vi "Initialize.vi"(6 "Filter":T1 {"Deny List (ID)" format="%.0x"; "Allow List (ID)" format="%.0x"}, 7 "Use OS Timestamp":bool, 8 "error in (no error)":errorcluster, 9 "Port Configuration":T2={"Mode"=enum."CAN FD", "Baud Rate"=500000, "Temination On"=TRUE, "Subordinate"=FALSE, "Echo TX"=FALSE, "FD Config"={"FD Baud Rate"=2000000, "ISO Mode"=TRUE, "BRS Enabled"=TRUE}} {"FD Config"."FD Baud Rate" format="%.0p"; "Baud Rate" format="%.0p"}, 10 "Interface":string, 11 "XNET_CAN_RW in":refnum<class "XNET CAN RW.lvclass">) -> (0 "error out":errorcluster, 3 "XNET_CAN_RW out":refnum<class "XNET CAN RW.lvclass">)   [LabVIEW 2021, in "XNET CAN RW.lvclass"]
doc: "Initialize a CAN read or write session using NI XNET hardware. \n\nInterface is the name of the XNET interface (eg CAN1)\n\nPort configuration sets the details of the CAN communication. Subordinate indicates another session has already configured the CAN port and this should use those settings.\n\nFilter provides a mecahnism to allow (white list) and deny (black list) certain ID from being returned or output. \n\nUse OS Timestamp will cause a read to replace the timestamp from the CAN driver with a timestamp from the OS. This is useful for correlation to othe events on the OS since the CAN clock will drift from the OS clock."
uses:
  XNET CAN RW.lvclass
  C:/Program Files/National Instruments/LabVIEW 2021/vi.lib/CIF Foundation/CIF CAN RW Core/CAN_RW_CORE.lvclass
  <vilib>/CIF Foundation/CIF CAN RW Core/typedef/CAN Port Configuration.ctl
  <vilib>/CIF Foundation/CIF CAN RW Core/typedef/CAN Mode.ctl
  <vilib>/CIF Foundation/CIF CAN RW Core/typedef/FD Config.ctl
  <vilib>/CIF Foundation/CIF CAN RW Core/typedef/CAN Filter.ctl
  XNET CAN RW.lvclass/XNET CAN RW.ctl
  <vilib>/CIF Foundation/CIF CAN RW Core/CAN_RW_CORE.lvclass
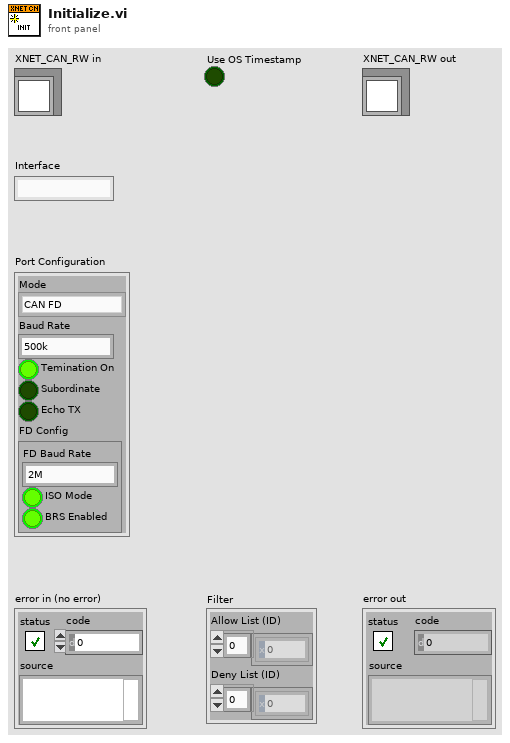
[diagram p1: front panel]
types:
  T1 = typedef "CAN_RW_CORE.lvclass/CAN Filter.ctl" = cluster{"Allow List (ID)":u32[], "Deny List (ID)":u32[]}
  T2 = typedef "CAN_RW_CORE.lvclass/CAN Port Configuration.ctl" = cluster{"Mode":T3, "Baud Rate":u64, "Temination On":bool, "Subordinate":bool, "Echo TX":bool, "FD Config":T4}
  T3 = typedef "CAN_RW_CORE.lvclass/CAN Mode.ctl" = enum16{"CAN 2.0", "CAN FD"}
  T4 = typedef "CAN_RW_CORE.lvclass/FD Config.ctl" = cluster{"FD Baud Rate":u64, "ISO Mode":bool, "BRS Enabled":bool}
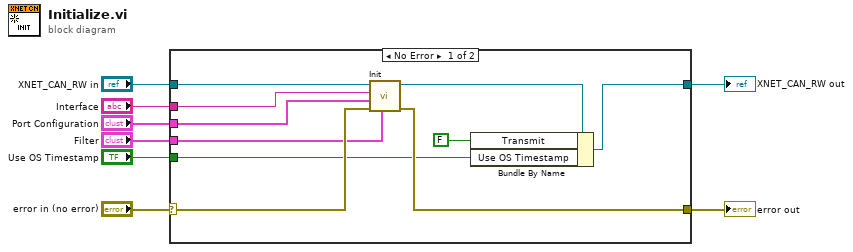
[diagram p0: block diagram]
diagram:
  n1 = case shown="No Error" "error in (no error)" {
    selector: "error in (no error)" -> [w13 w20]
    tunnel: [w11 w20] -> w7
    tunnel: [w18 w19] -> w5
    tunnel: "XNET_CAN_RW in" -> [w16 w19]
    tunnel: "Interface" -> [w15 _]
    tunnel: "Port Configuration" -> [w14 _]
    tunnel: "Filter" -> [w12 _]
    tunnel: "Use OS Timestamp" -> [w9 _]
    frame No Error {
      n2 = call <vilib>:"Init.vi"("Filter"=w12, "error in (no error)"=w13, "Port Configuration"=w14, "Interface"=w15, "CAN_RW_CORE in"=w16) -> ("error out"=w11:errorcluster, "CAN_RW_CORE out"=w10:refnum<class "XNET CAN RW.lvclass">)  [unwired: 5 in]
      n3 = Bundle By Name(cluster=w10, "Transmit"=FALSE, "Use OS Timestamp"=w9) -> (w18:refnum<class "XNET CAN RW.lvclass">)
    }
    frame Error {
    }
  }
  "error out" <- w7
  "XNET_CAN_RW out" <- w5
